vi "3. Message Helper VI and Equivalent String.vi"() -> ()   [LabVIEW 2017]
doc: "#### Overview\n\nDemonstrates the string syntax format for message communication within the CSM framework.\n\n#### Introduction\n\nThis example explains the syntax format for inter-module message communication in CSM. You can use LabVIEW APIs to build these strings. If you are familiar with the message rules, you can create them manually. The syntax defined by CSM is as follows:\n\n```\n //--- CSM State Syntax ---\n // Local Message Example\n DoSth: DoA >> Arguments\n\n // Synchronous Call Example\n API: xxxx >> Arguments -@ TargetModule\n\n // Asynchronous Call Example\n API: xxxx >> Arguments -> TargetModule\n\n // Asynchronous Call (No Reply) Example\n API: xxxx >> Arguments ->| TargetModule\n\n // Broadcast Normal Status:\n Status >> StatusArguments -><status>\n\n // Broadcast Interrupt Status:\n Interrupt >> StatusArguments -><interrupt>\n\n // Register Source Module's State to Handler Module\n Status@Source Module >> API@Handler Module -><register>\n\n // Unregister Source Module's State\n Status@Source Module >> API@Handler Module -><unregister>\n\n //--- CSM Comments ---\n // To add a comment, use \"//\". All text to the right will be ignored.\n UI: Initialize // Initialize UI\n // Another comment line\n```\n\n#### Steps\n\n- Step1: Synchronous message. The sender waits in place for a reply until a timeout occurs or a reply is received.\n- Step2: Asynchronous message with reply. The sender continues to execute subsequent operations without waiting for a reply. After the receiver processes the message, it replies to the sender.\n- Step3: Asynchronous message without reply. The sender continues to execute subsequent operations without waiting for a reply. After the receiver processes the message, it does not reply to the sender.\n- Step4: Broadcast a normal status string.\n- Step5: Broadcast an interrupt or high-priority status string.\n- Step6: Register a state. When the state changes, the registered handler module message is automatically triggered.\n- Step7: Unregister a state. Cancels the message trigger upon state change."
uses:
  user.lib/_NEVSTOP/Communicable State Machine(CSM)/_Polymophic/Build Synchronous Message with Arguments.vi
  user.lib/_NEVSTOP/Communicable State Machine(CSM)/_Polymophic/Build Asynchronous Message with Arguments.vi
  user.lib/_NEVSTOP/Communicable State Machine(CSM)/_Polymophic/Build Interrupt Broadcast Message.vi
  user.lib/_NEVSTOP/Communicable State Machine(CSM)/_Polymophic/Build No-Reply Asynchronous Message with Arguments.vi
  user.lib/_NEVSTOP/Communicable State Machine(CSM)/_Polymophic/Build Unregister Message.vi
  user.lib/_NEVSTOP/Communicable State Machine(CSM)/_Polymophic/Build Register Message.vi
  user.lib/_NEVSTOP/Communicable State Machine(CSM)/Communicable State Machine.lvlib
panel:
  out "Equivalent String (Register Status)":string="Status Changed-> <all>"
  out "Equivalent String (Unregister Status)":string="Status Changed >> Argument-> <all>"
  out "Equivalent String (Async without reply Message)":string="State >> Argument->DestModuleName"
  out "Equivalent String (Interrupt Status)":string="Status Changed >> Argument-> <all>"
  out "Equivalent String (Normal Status)":string="Status Changed-> <all>"
  out "Equivalent String (Async Message)":string="State >> Argument->DestModuleName"
  out "Equivalent String (Sync Message)":string="State >> Argument@DestModuleName"
  # "#CSM-Example Overview\n\nDemonstrates the string syntax format for message communication within the CSM framework."
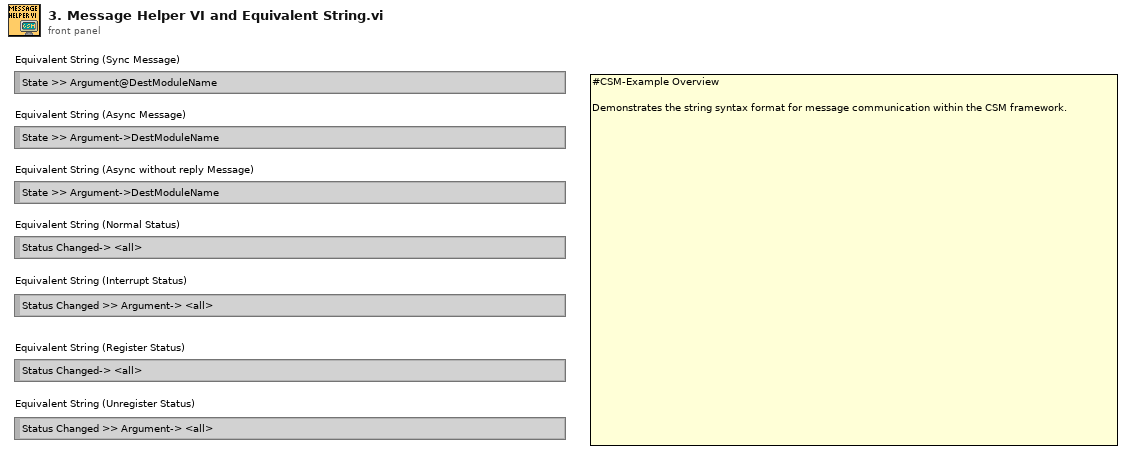
[diagram p1: front panel]
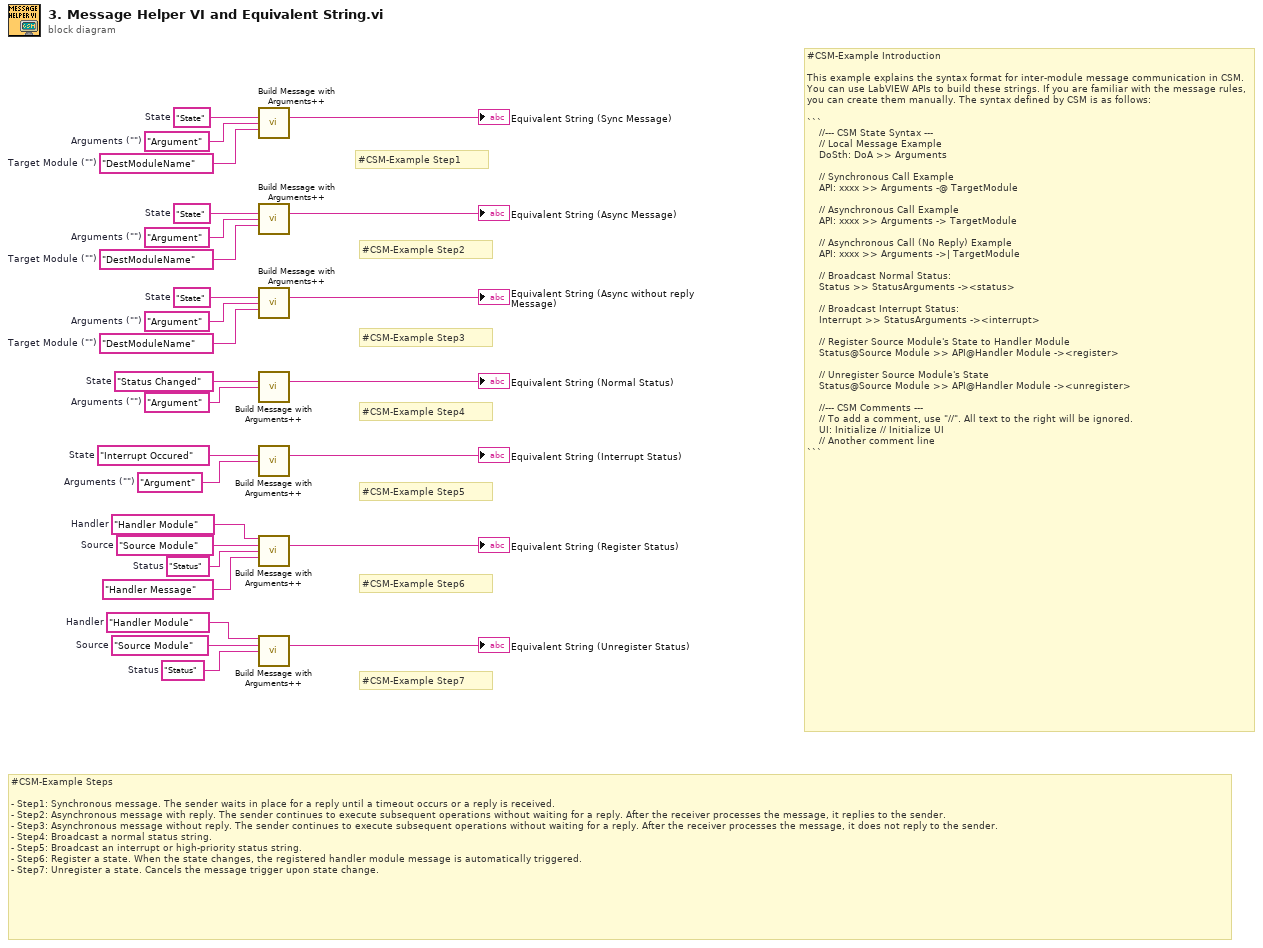
[diagram p0: block diagram]
diagram:
  w2 = "Handler Module"  # Handler
  w3 = "Handler Module"  # Handler
  w9 = "Status"  # Status
  w7 = "Status"  # Status
  w6 = "Source Module"  # Source
  w8 = "Source Module"  # Source
  w10 = "Argument"  # Arguments ("")
  w16 = "Argument"  # Arguments ("")
  w15 = "DestModuleName"  # Target Module ("")
  w17 = "State"  # State
  w12 = "Argument"  # Arguments ("")
  w13 = "Interrupt Occured"  # State
  w11 = "Status Changed"  # State
  w21 = "Argument"  # Arguments ("")
  w22 = "DestModuleName"  # Target Module ("")
  w20 = "State"  # State
  w26 = "Argument"  # Arguments ("")
  w25 = "DestModuleName"  # Target Module ("")
  w27 = "State"  # State
  # "#CSM-Example Step7"
  # "#CSM-Example Step6"
  # "#CSM-Example Step5"
  # "#CSM-Example Step4"
  # "#CSM-Example Step3"
  # "#CSM-Example Step2"
  # "#CSM-Example Step1"
  # "#CSM-Example Steps\n\n- Step1: Synchronous message. The sender waits in place for a reply until a timeout occurs or a reply is received.\n- Step2: Asynchronous message with reply. The sender continues to execute subsequent operations without waiting for a reply. After the receiver processes the message, it replies to the sender.\n- Step3: Asynchronous message without reply. The sender continues to execute subsequent operations without waiting for a reply. After the receiver processes the message, it does not reply to the sender.\n- Step4: Broadcast a normal status string.\n- Step5: Broadcast an interrupt or high-priority status string.\n- Step6: Register a state. When the state changes, the registered handler module message is automatically triggered.\n- Step7: Unregister a state. Cancels the message trigger upon state change."
  # "#CSM-Example Introduction\n\nThis example explains the syntax format for inter-module message communication in CSM. You can use LabVIEW APIs to build these strings. If you are familiar with the message rules, you can create them manually. The syntax defined by CSM is as follows:\n\n```\n    //--- CSM State Syntax ---\n    // Local Message Example\n    DoSth: DoA >> Arguments\n\n    // Synchronous Call Example\n    API: xxxx >> Arguments -@ TargetModule\n\n    // Asynchronous Call Example\n    API: xxxx >> Arguments -> TargetModule\n\n    // Asynchronous Call (No Reply) Example\n    API: xxxx >> Arguments ->| TargetModule\n\n    // Broadcast Normal Status:\n    Status >> StatusArguments -><status>\n\n    // Broadcast Interrupt Status:\n    Interrupt >> StatusArguments -><interrupt>\n\n    // Register Source Module's State to Handler Module\n    Status@Source Module >> API@Handler Module -><register>\n\n    // Unregister Source Module's State\n    Status@Source Module >> API@Handler Module -><unregister>\n\n    //--- CSM Comments ---\n    // To add a comment, use \"//\". All text to the right will be ignored.\n    UI: Initialize // Initialize UI\n    // Another comment line\n```"
  n1 = call-poly "Build Message with Arguments++.vi"("State With Arguments"=w27, "Arguments (\"\")"=w26, "Target Module (\"\")"=w25) -> ("CSM Message String"=→"Equivalent String (Sync Message)":string)  [unwired: 12 in]
  n2 = call-poly "Build Message with Arguments++.vi"("State With Arguments"=w20, "Arguments (\"\")"=w21, "Target Module (\"\")"=w22) -> ("CSM Message String"=→"Equivalent String (Async Message)":string)  [unwired: 12 in]
  n3 = call-poly "Build Message with Arguments++.vi"("State With Arguments"=w17, "Arguments (\"\")"=w16, "Target Module (\"\")"=w15) -> ("CSM Message String"=→"Equivalent String (Async without reply Message)":string)  [unwired: 12 in]
  n4 = call-poly "Build Message with Arguments++.vi"("Source CSM (* as Default)"=w11, "Status"=w10) -> ("CSM Message String"=→"Equivalent String (Normal Status)":string)  [unwired: 13 in]
  n5 = call-poly "Build Message with Arguments++.vi"("State With Arguments"=w13, "Arguments (\"\")"=w12) -> ("CSM Message String"=→"Equivalent String (Interrupt Status)":string)  [unwired: 13 in]
  n6 = call-poly "Build Message with Arguments++.vi"("Target CSM"=w2, "Source CSM (* as Default)"=w8, "Status"=w9, "API (If \"\", Same As \"Status\")"="Handler Message" ("Response Message (if \"\", same as Source Message)")) -> ("CSM Message String"=→"Equivalent String (Register Status)":string)  [unwired: 11 in]
  n7 = call-poly "Build Message with Arguments++.vi"("Target CSM"=w3, "Source CSM (* as Default)"=w6, "Status"=w7) -> ("CSM Message String"=→"Equivalent String (Unregister Status)":string)  [unwired: 12 in]
